vi "SpO2_Processing.vi"() -> ()   [LabVIEW 2018]
uses:
  <vilib>/Analysis/3filter.llb/Filter Passband Type.ctl
  <vilib>/Analysis/1siggen.llb/Ramp Pattern by Samples.vi
  <vilib>/Utility/file.llb/Read Delimited Spreadsheet (DBL).vi
  <vilib>/Analysis/3filter.llb/Butterworth Filter (DBL).vi
  <vilib>/Analysis/NI_AALBase.lvlib
  <vilib>/Analysis/NI_AAL_SigProc.lvlib
  <vilib>/Analysis/NI_AALPro.lvlib
panel:
  out "dX/dt":dbl[](array[numeric])
  out "x/y":dbl[](array[numeric])
  out "IR PPG":cluster{dbl[], dbl[]}[](graph) caption="Raw PPG"
  in  "IR Peak Threshold":dbl step=0.001 format="%0.3f"
  in  "IR Width":i32=3 min=3
  in  "IR Valley Threshold":dbl step=0.001 format="%0.3f"
  in  "Red Valley Threshold":dbl step=0.001 format="%0.3f"
  in  "Red Width":i32=3 min=3
  in  "Red Peak Threshold":dbl step=0.001 format="%0.3f"
  out "Raw PPG 2":cluster{dbl[], dbl[]}[](graph) caption="Raw PPG"
  in  "Interval (s)":dbl
  in  "Begin (s)":dbl
  out "Raw PPG":cluster{dbl[], dbl[]}[](graph)
  in  "Sampling Frequency(Hz)":dbl=500.0
  in  "File Path":path
  # "Raw PPG"
  # "Red PPG"
  # "IR PPG"
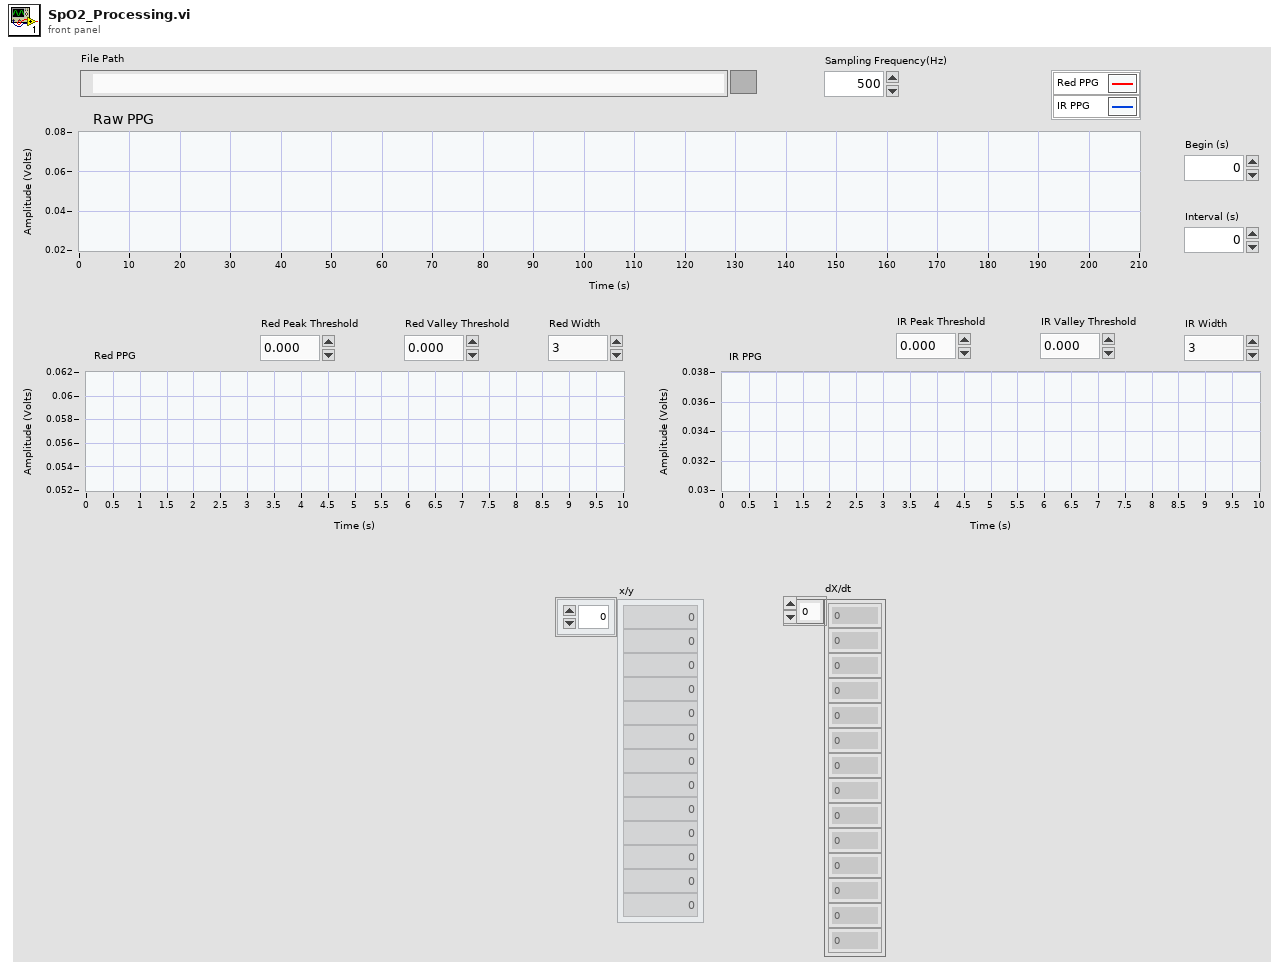
[diagram p1: front panel]
types:
  T1 = typedef "NI_AALBase.lvlib/Filter Passband Type.ctl" = enum32{"Lowpass", "Highpass", "Bandpass", "Bandstop"}
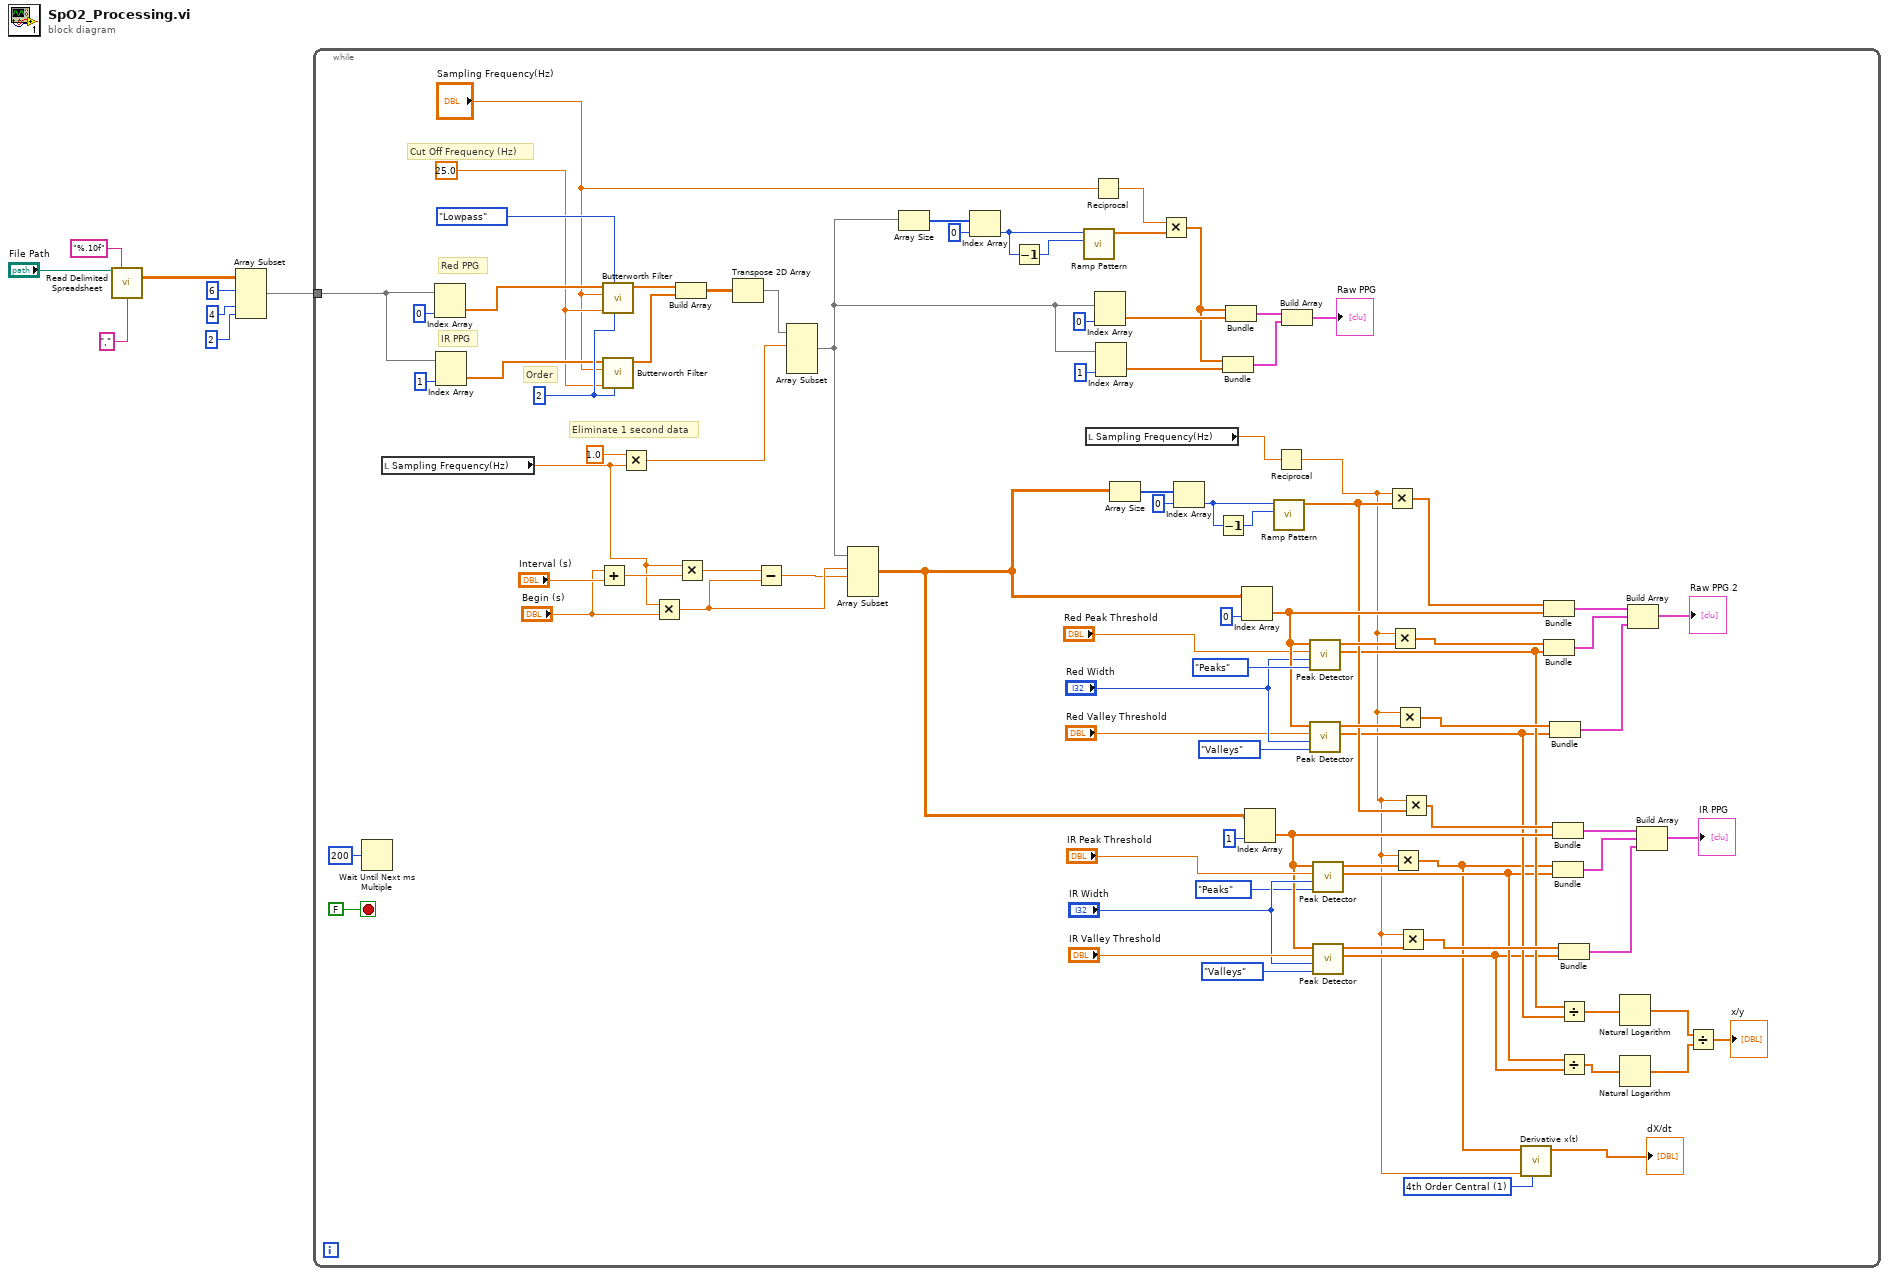
[diagram p0: block diagram]
diagram:
  n1 = call-poly <vilib>:"Read Delimited Spreadsheet.vi"("file path (dialog if empty)"="File Path", "format (%.3f)"="%.10f", "delimiter (\\t)"=",") -> ("all rows"=w5:dbl[][])  [unwired: 7 in, 5 out]
  n2 = Array Subset(array=w5, index (row)=6 ("index"), index (col)=4 ("disabled index (col)"), length (col)=2 ("disabled index (col)")) -> (w1:dbl[][])  [unwired: 1 in]
  n3 = while {
    tunnel: w1 -> [w95]
    stop <- FALSE stop-if-true
    w10 = u16 1 items=["2nd Order Central", "4th Order Central", "Forward", "Backward"] ("method")
    w91 = 25.0 ("Cutoff Frequency(Hz)")
    w93 = 2 ("order")
    # "Cut Off Frequency (Hz)"
    # "Eliminate 1 second data"
    # "IR PPG"
    # "Red PPG"
    # "Order"
    n4 = Wait Until Next ms Multiple(millisecond multiple=u32 200) -> ()  [unwired: 1 out]
    n5 = local read "Sampling Frequency(Hz)"() -> (w54:dbl)
    n6 = Index Array(array=w95, index (col)=0 ("disabled index (col)")) -> (element=w94:dbl[])  [unwired: 1 in]
    n7 = Index Array(array=w95, index (col)=1 ("disabled index (col)")) -> (element=w92:dbl[])  [unwired: 1 in]
    n8 = Add(x="Begin (s)", y="Interval (s)") -> (x+y=w57:dbl)
    n9 = call-poly <vilib>:"Butterworth Filter.vi"("order"=w93, "filter type"=Filter_Passband_Type."Lowpass", "low cutoff freq: fl"=w91, "sampling freq: fs"="Sampling Frequency(Hz)", "X"=w94) -> ("Filtered X"=w90:dbl[])  [unwired: 3 in, 1 out]
    n10 = call-poly <vilib>:"Butterworth Filter.vi"("order"=w93, "low cutoff freq: fl"=w91, "sampling freq: fs"="Sampling Frequency(Hz)", "X"=w92) -> ("Filtered X"=w89:dbl[])  [unwired: 4 in, 1 out]
    n11 = Multiply(x=1.0, y=w54) -> (x*y=w60:dbl)
    n12 = Multiply(x=w54, y="Begin (s)") -> (x*y=w69:dbl)
    n13 = Build Array(w90, w89) -> (w88:dbl[][])
    n14 = Multiply(x=w54, y=w57) -> (x*y=w70:dbl)
    n15 = Transpose 2D Array(2D array=w88) -> (transposed array=w87:dbl[][])
    n16 = Subtract(x=w70, y=w69) -> (x-y=w56:dbl)
    n17 = Array Subset(array=w87, index (row)=w60) -> (w71:dbl[][])  [unwired: 3 in]
    n18 = Array Subset(array=w71, index (row)=w69, length (row)=w56) -> (w25:dbl[][])  [unwired: 2 in]
    n19 = Array Size(array=w71) -> (size(s)=w86:i32[])
    n20 = Index Array(array=w86, index=0) -> (element=w84:i32)
    n21 = Decrement(x=w84) -> (x-1=w83:i32)
    n22 = call-poly <vilib>:"Ramp Pattern.vi"("end"=w83, "samples"=w84) -> ("Ramp Pattern"=w82:dbl[])  [unwired: 8 in, 1 out]
    n23 = local read "Sampling Frequency(Hz)"() -> (w39:dbl)
    n24 = Reciprocal(x="Sampling Frequency(Hz)") -> (1/x=w76:dbl)
    n25 = Index Array(array=w71, index (col)=0 ("disabled index (col)")) -> (element=w77:dbl[])  [unwired: 1 in]
    n26 = Index Array(array=w71, index (col)=1) -> (element=w73:dbl[])  [unwired: 1 in]
    n27 = Array Size(array=w25) -> (size(s)=w61:i32[])
    n28 = Multiply(x=w76, y=w82) -> (x*y=w75:dbl[])
    n29 = Index Array(array=w61, index=0) -> (element=w63:i32)
    n30 = Decrement(x=w63) -> (x-1=w64:i32)
    n31 = Bundle(w75, w73) -> (w72:cluster{dbl[], dbl[]})  [unwired: 1 in]
    n32 = Bundle(w75, w77) -> (w79:cluster{dbl[], dbl[]})  [unwired: 1 in]
    n33 = Index Array(array=w25, index (col)=0 ("disabled index (col)")) -> (element=w46:dbl[])  [unwired: 1 in]
    n34 = Index Array(array=w25, index (col)=1 ("disabled index (col)")) -> (element=w34:dbl[])  [unwired: 1 in]
    n35 = call-poly <vilib>:"Ramp Pattern.vi"("end"=w64, "samples"=w63) -> ("Ramp Pattern"=w24:dbl[])  [unwired: 8 in, 1 out]
    n36 = Reciprocal(x=w39) -> (1/x=w11:dbl)
    n37 = Build Array(w79, w72) -> (→"Raw PPG":cluster{dbl[], dbl[]}[])
    n38 = call <vilib>:"Peak Detector.vi"("peaks/valleys"=enum32{"Peaks", "Valleys"}."Peaks", "width"="Red Width", "threshold"="Red Peak Threshold", "X"=w46) -> ("Amplitudes"=w21:dbl[], "Locations"=w50:dbl[])  [unwired: 3 in, 3 out]
    n39 = call <vilib>:"Peak Detector.vi"("peaks/valleys"=enum32{"Peaks", "Valleys"}."Valleys", "width"="Red Width", "threshold"="Red Valley Threshold", "X"=w46) -> ("Amplitudes"=w20:dbl[], "Locations"=w41:dbl[])  [unwired: 3 in, 3 out]
    n40 = call <vilib>:"Peak Detector.vi"("peaks/valleys"=enum32{"Peaks", "Valleys"}."Peaks", "width"="IR Width", "threshold"="IR Peak Threshold", "X"=w34) -> ("Amplitudes"=w18:dbl[], "Locations"=w31:dbl[])  [unwired: 3 in, 3 out]
    n41 = call <vilib>:"Peak Detector.vi"("peaks/valleys"=enum32{"Peaks", "Valleys"}."Valleys", "width"="IR Width", "threshold"="IR Valley Threshold", "X"=w34) -> ("Amplitudes"=w17:dbl[], "Locations"=w23:dbl[])  [unwired: 3 in, 3 out]
    n42 = Multiply(x=w11, y=w24) -> (x*y=w68:dbl[])
    n43 = Multiply(x=w11, y=w50) -> (x*y=w49:dbl[])
    n44 = Multiply(x=w11, y=w31) -> (x*y=w12:dbl[])
    n45 = Multiply(x=w11, y=w41) -> (x*y=w43:dbl[])
    n46 = Multiply(x=w11, y=w23) -> (x*y=w37:dbl[])
    n47 = Multiply(x=w11, y=w24) -> (x*y=w26:dbl[])
    n48 = call <vilib>:"Derivative x(t).vi"("method"=w10, "dt"=w11, "X"=w12) -> ("dX/dt"=→"dX/dt":dbl[])  [unwired: 7 in, 1 out]
    n49 = Bundle(w68, w46) -> (w66:cluster{dbl[], dbl[]})  [unwired: 1 in]
    n50 = Bundle(w49, "Amplitudes"=w21) -> (w48:cluster{dbl[], "Amplitudes":dbl[]})  [unwired: 1 in]
    n51 = Bundle(w43, "Amplitudes"=w20) -> (w42:cluster{dbl[], "Amplitudes":dbl[]})  [unwired: 1 in]
    n52 = Bundle(w26, w34) -> (w28:cluster{dbl[], dbl[]})  [unwired: 1 in]
    n53 = Bundle(w12, "Amplitudes"=w18) -> (w32:cluster{dbl[], "Amplitudes":dbl[]})  [unwired: 1 in]
    n54 = Bundle(w37, "Amplitudes"=w17) -> (w22:cluster{dbl[], "Amplitudes":dbl[]})  [unwired: 1 in]
    n55 = Divide(x=w21, y=w20) -> (x/y=w19:dbl[])
    n56 = Divide(x=w18, y=w17) -> (x/y=w16:dbl[])
    n57 = Natural Logarithm(1:w19) -> (0:w15:dbl[])
    n58 = Natural Logarithm(1:w16) -> (0:w14:dbl[])
    n59 = Build Array(w66, w48, w42) -> (→"Raw PPG 2":cluster{dbl[], "Amplitudes":dbl[]}[])
    n60 = Build Array(w28, w32, w22) -> (→"IR PPG":cluster{dbl[], "Amplitudes":dbl[]}[])
    n61 = Divide(x=w15, y=w14) -> (x/y=→"x/y":dbl[])
  }
